vi "FAHRENHEIT_A_CELSIUS.vi"() -> ()   [LabVIEW 2026]
panel:
  out "°C":dbl
  in  "°F":dbl
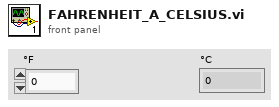
[diagram p1: front panel]
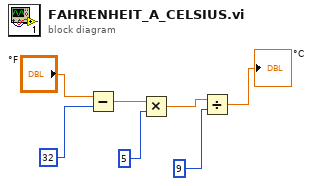
[diagram p0: block diagram]
diagram:
  n1 = Subtract(x="°F", y=32) -> (x-y=w5:dbl)
  n2 = Multiply(x=w5, y=5) -> (x*y=w2:dbl)
  n3 = Divide(x=w2, y=9) -> (x/y=→"°C":dbl)
